vi "Lidar_Machine_etats.vi"() -> ()   [LabVIEW 2018]
uses:
  enum_etats_lidar.ctl
  <vilib>/Platform/TimedLoop/XDataNode/timing_clust.ctl
  <vilib>/Platform/TimedLoop/XDataNode/nitl_modes.ctl
  <vilib>/Platform/TimedLoop/XDataNode/wakeup.ctl
  enum_zone.ctl
  <vilib>/Platform/TimedLoop/XDataNode/XDataNode.xnode
  <vilib>/Platform/TimedLoop/XDataNode/XDNodeRunTimeDep.lvlib
panel:
  out "error boucle cadencé":errorcluster
  out "error boucle principale":errorcluster
  out "Espace libre":dbl[][](array[numeric])
  out "Zone 3":dbl[][](array[numeric])
  out "Zone 2":dbl[][](array[numeric])
  out "Timeout":bool=TRUE
  out "Selection de état":T1
  in  "stop boucle cadencé":bool
  out "Tableau lidar":dbl[][](array[numeric])=[[0.0, 1.0, 2.0, 3.0, 4.0, 5.0, 6.0, 7.0, 8.0, 9.0, 10.0, 11.0, 12.0, 13.0, 14.0, 15.0, 16.0, 17.0, 18.0, 19.0, 20.0, 21.0, 22.0, 23.0, 24.0, 25.0, 26.0, 27.0, 28.0, 29.0, 30.0, 31.0, 32.0, 33.0, 34.0, 35.0], [20.0, 15.0, 30.0, 31.0, 42.0, 50.0, 51.0, 60.0, 20.0, 15.0, 30.0, 31.0, 42.0, 50.0, 51.0, 60.0, 20.0, 15.0, 30.0, 31.0, 42.0, 50.0, 51.0, 60.0, 20.0, 15.0, 30.0, 31.0, 42.0, 50.0, 51.0, 60.0, 20.0, 15.0, 30.0, 31.0], [0.0, 0.0, 0.0, 0.0, 0.0, 0.0, 0.0, 0.0, 0.0, 0.0, 0.0, 0.0, 0.0, 0.0, 0.0, 0.0, 0.0, 0.0, 0.0, 0.0, 0.0, 0.0, 0.0, 0.0, 0.0, 0.0, 0.0, 0.0, 0.0, 0.0, 0.0, 0.0, 0.0, 0.0, 0.0, 0.0]]
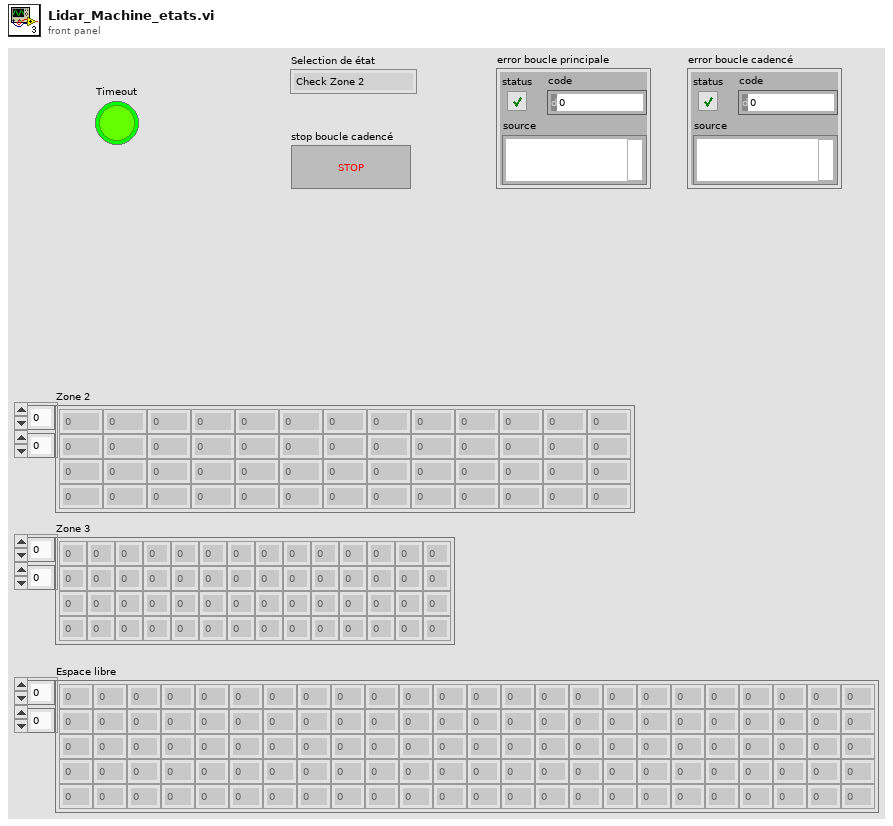
[diagram p1: front panel]
types:
  T1 = typedef "enum_etats_lidar.ctl" = enum16{"Check Zone 2", "Obstacle Zone 2", "Check Zone 3", "Obstacle Zone 3", "Avance", "Obstacle Timer", "Rescan 10s", "Check Zone 3 Bis", "Rotation new direction", "Rotation 180", "Timeout ?", "Arret complet", "Rotation new dir timer", "Rotation 180 timer"}
  T2 = typedef "enum_zone.ctl" = enum16{"Zone_2", "Zone_3", "Espace_libre", "Aucune"}
  T3 = typedef "XDNodeRunTimeDep.lvlib/timing_clust.ctl" = cluster{"Expected End [f-1]":u64, "Actual End [f-1]":u64, "Finished Late? [f-1]":bool, "Expected End [i-1]":u64, "Actual End [i-1]":u64, "Finished Late? [i-1]":bool, "Expected Start [i]":u64, "Actual Start [i]":u64, "Expected Start [f]":u64, "Actual Start [f]":u64, "Source Name":string, "Structure Name":string, "Period":i64, "Deadline":i64, "Offset":i64, "Start":i64, "Priority":i32, "Timeout":i32, "Mode":T4, "Wakeup Reason":T5, "Error":errorcluster, "Source Type":string, "Secondary Source Type":string, "Global End Time":u64, "Global Start Time":u64, "Frame Duration":u64, "Iteration Duration":u64, "Assigned CPU":i32, "I/O Scan Engine Mode":u32}
  T4 = typedef "XDNodeRunTimeDep.lvlib/nitl_modes.ctl" = enum32{"No Change", "Process missed periods, maintain original phase", "Discard missed periods, maintain original phase", "Process missed periods, ignore original phase", "Discard missed periods, ignore original phase"}
  T5 = typedef "XDNodeRunTimeDep.lvlib/wakeup.ctl" = enum32{"Normal", "Aborted", "Asynchronous wakeup", "Timing source error", "Timed loop error", "Timeout"}
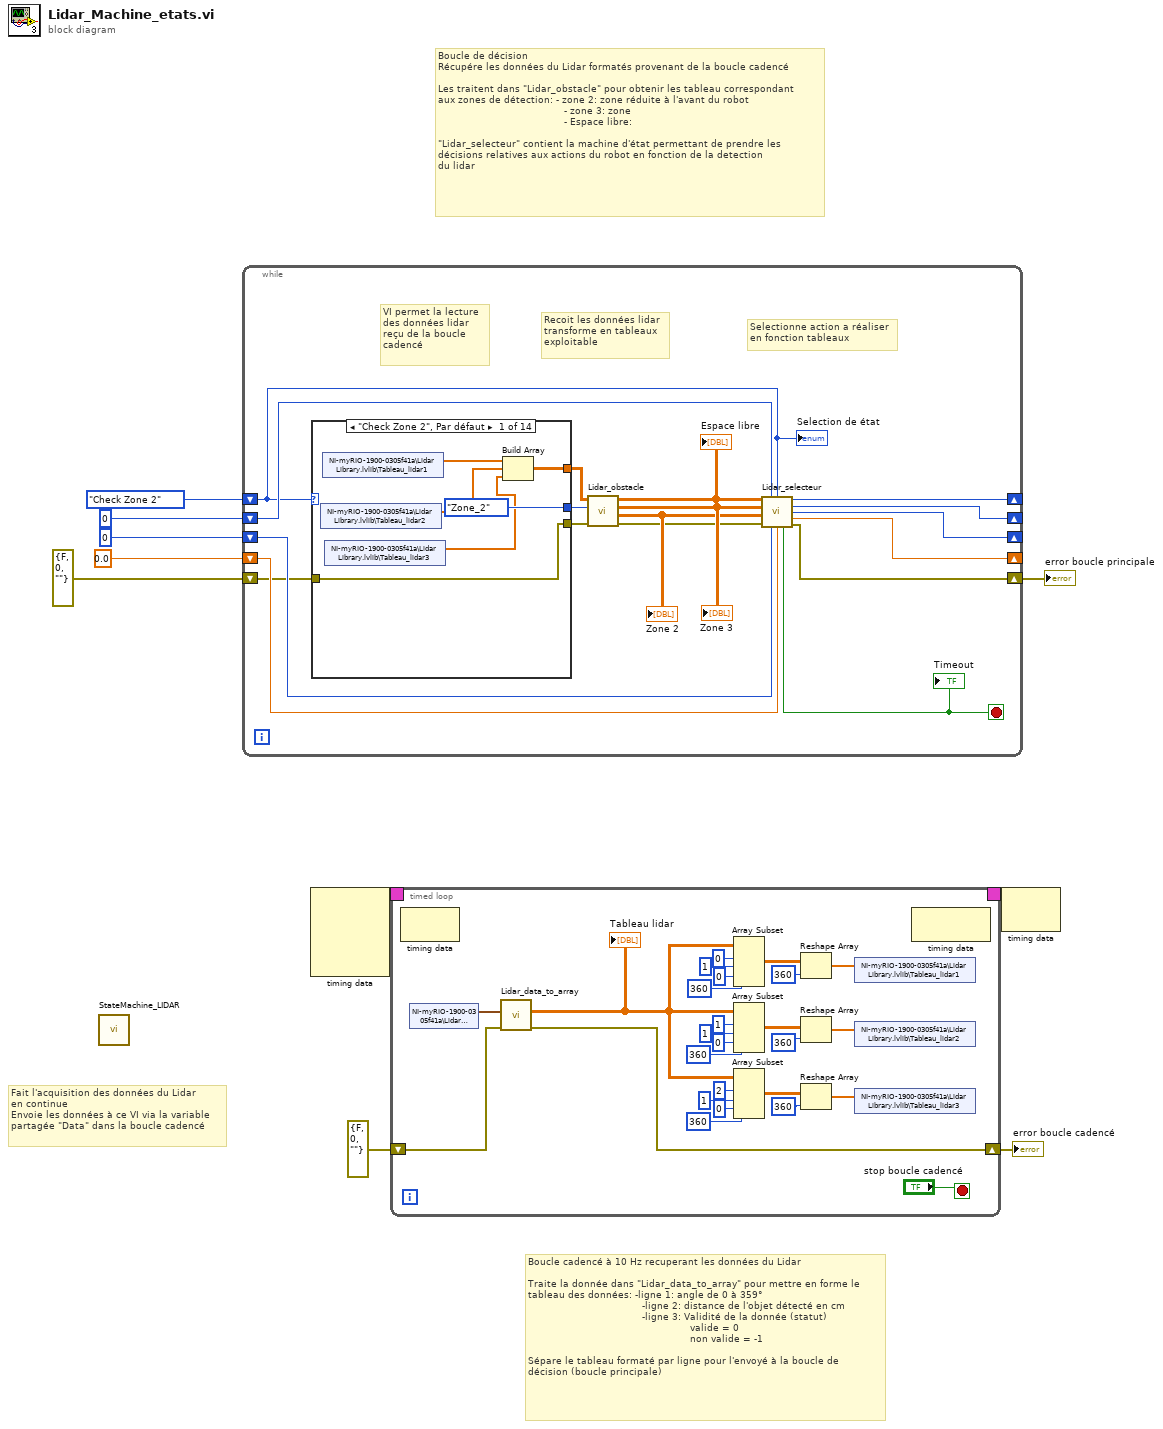
[diagram p0: block diagram]
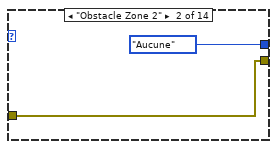
[diagram p2: hidden frame]
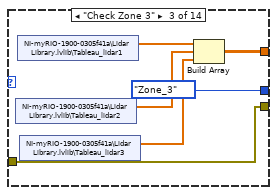
[diagram p3: hidden frame]
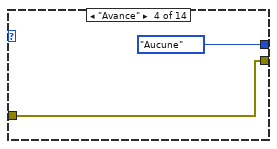
[diagram p4: hidden frame]
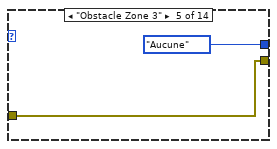
[diagram p5: hidden frame]
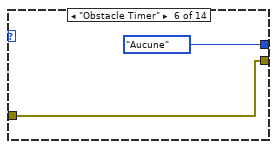
[diagram p6: hidden frame]
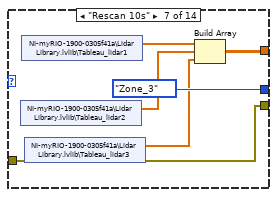
[diagram p7: hidden frame]
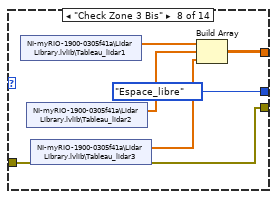
[diagram p8: hidden frame]
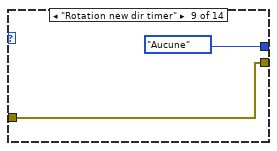
[diagram p9: hidden frame]
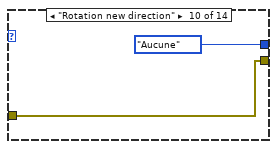
[diagram p10: hidden frame]
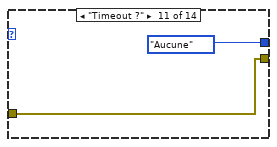
[diagram p11: hidden frame]
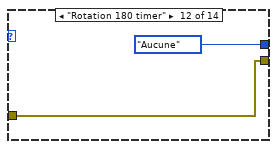
[diagram p12: hidden frame]
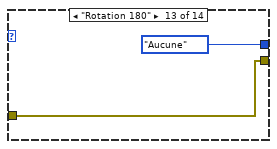
[diagram p13: hidden frame]
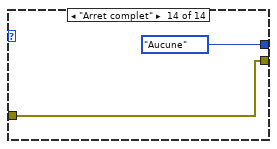
[diagram p14: hidden frame]
diagram:
  # "Boucle de décision\nRécupére les données du Lidar formatés provenant de la boucle cadencé\n\nLes traitent dans \"Lidar_obstacle\" pour obtenir les tableau correspondant \naux zones de détection: - zone 2: zone réduite à l'avant du robot\n                                          - zone 3: zone \n                                          - Espace libre: \n\n\"Lidar_selecteur\" contient la machine d'état permettant de prendre les\ndécisions relatives aux actions du robot en fonction de la detection\ndu lidar"
  # "Boucle cadencé à 10 Hz recuperant les données du Lidar\n\nTraite la donnée dans \"Lidar_data_to_array\" pour mettre en forme le\ntableau des données: -ligne 1: angle de 0 à 359°\n                                      -ligne 2: distance de l'objet détecté en cm\n                                      -ligne 3: Validité de la donnée (statut)\n                                                      valide = 0\n                                                      non valide = -1\n\nSépare le tableau formaté par ligne pour l'envoyé à la boucle de\ndécision (boucle principale)"
  # "Fait l'acquisition des données du Lidar\nen continue\nEnvoie les données à ce VI via la variable \npartagée \"Data\" dans la boucle cadencé"
  n1 = call "StateMachine_LIDAR.vi"() -> ()  [unwired: 12 in]
  n2 = while {
    shift-right: [w24] -> _
    shift-left: enum_etats_lidar."Check Zone 2" ("Selection de état") -> [w15]
    shift-right: [w22] -> _
    shift-left: u32 0 ("Timeout Count") -> [w23]
    shift-right: [w21] -> _
    shift-left: u32 0 ("Tick Count(mSec)") -> [w20]
    shift-right: [w18] -> _
    shift-left: 0.0 ("New Angle") -> [w19]
    shift-right: [w16] -> w2
    shift-left: errorcluster {"status"=FALSE, "code"=0, "source"=""} ("error out") -> [w13]
    stop <- w17 stop-if-true
    # "VI permet la lecture \ndes données lidar\nreçu de la boucle\ncadencé"
    # "Selectionne action a réaliser\nen fonction tableaux"
    # "Recoit les données lidar\ntransforme en tableaux \nexploitable"
    n3 = case shown="\"Check Zone 2\", Par défaut" w15 {
      tunnel: [enum_zone."Zone_2" ("Enum Zone") enum_zone."Aucune" ("Enum Zone") enum_zone."Zone_3" ("Enum Zone") enum_zone."Aucune" ("Enum Zone") enum_zone."Aucune" ("Enum Zone") enum_zone."Aucune" ("Enum Zone") enum_zone."Zone_3" ("Enum Zone") enum_zone."Espace_libre" ("Enum Zone") enum_zone."Aucune" ("Enum Zone") enum_zone."Aucune" ("Enum Zone") enum_zone."Aucune" ("Enum Zone") enum_zone."Aucune" ("Enum Zone") enum_zone."Aucune" ("Enum Zone") enum_zone."Aucune" ("Enum Zone")] -> w14
      tunnel: w13 -> [w33 w35 w41 w43 w45 w47 w53 w59 w61 w63 w65 w67 w69 w71]
      tunnel: [w33 w35 w41 w43 w45 w47 w53 w59 w61 w63 w65 w67 w69 w71] -> w12
      tunnel: [w29 _ w37 _ _ _ w52 w58 _ _ _ _ _ _] -> w11
      frame "Check Zone 2", Default {
        n4 = shared-variable "NI-myRIO-1900-0305f41a\\Lidar Library.lvlib\\Tableau_lidar2"() -> (w31:dbl[])  [unwired: 1 in, 1 out]
        n5 = shared-variable "NI-myRIO-1900-0305f41a\\Lidar Library.lvlib\\Tableau_lidar1"() -> (w32:dbl[])  [unwired: 1 in, 1 out]
        n6 = shared-variable "NI-myRIO-1900-0305f41a\\Lidar Library.lvlib\\Tableau_lidar3"() -> (w30:dbl[])  [unwired: 1 in, 1 out]
        n7 = Build Array(w32, w31, w30) -> (w29:dbl[][])
      }
      frame "Obstacle Zone 2" {
      }
      frame "Check Zone 3" {
        n8 = shared-variable "NI-myRIO-1900-0305f41a\\Lidar Library.lvlib\\Tableau_lidar2"() -> (w39:dbl[])  [unwired: 1 in, 1 out]
        n9 = shared-variable "NI-myRIO-1900-0305f41a\\Lidar Library.lvlib\\Tableau_lidar1"() -> (w40:dbl[])  [unwired: 1 in, 1 out]
        n10 = shared-variable "NI-myRIO-1900-0305f41a\\Lidar Library.lvlib\\Tableau_lidar3"() -> (w38:dbl[])  [unwired: 1 in, 1 out]
        n11 = Build Array(w40, w39, w38) -> (w37:dbl[][])
      }
      frame "Avance" {
      }
      frame "Obstacle Zone 3" {
      }
      frame "Obstacle Timer" {
      }
      frame "Rescan 10s" {
        n12 = shared-variable "NI-myRIO-1900-0305f41a\\Lidar Library.lvlib\\Tableau_lidar2"() -> (w50:dbl[])  [unwired: 1 in, 1 out]
        n13 = shared-variable "NI-myRIO-1900-0305f41a\\Lidar Library.lvlib\\Tableau_lidar1"() -> (w51:dbl[])  [unwired: 1 in, 1 out]
        n14 = shared-variable "NI-myRIO-1900-0305f41a\\Lidar Library.lvlib\\Tableau_lidar3"() -> (w49:dbl[])  [unwired: 1 in, 1 out]
        n15 = Build Array(w51, w50, w49) -> (w52:dbl[][])
      }
      frame "Check Zone 3 Bis" {
        n16 = shared-variable "NI-myRIO-1900-0305f41a\\Lidar Library.lvlib\\Tableau_lidar1"() -> (w57:dbl[])  [unwired: 1 in, 1 out]
        n17 = shared-variable "NI-myRIO-1900-0305f41a\\Lidar Library.lvlib\\Tableau_lidar2"() -> (w56:dbl[])  [unwired: 1 in, 1 out]
        n18 = shared-variable "NI-myRIO-1900-0305f41a\\Lidar Library.lvlib\\Tableau_lidar3"() -> (w55:dbl[])  [unwired: 1 in, 1 out]
        n19 = Build Array(w57, w56, w55) -> (w58:dbl[][])
      }
      frame "Rotation new dir timer" {
      }
      frame "Rotation new direction" {
      }
      frame "Timeout ?" {
      }
      frame "Rotation 180 timer" {
      }
      frame "Rotation 180" {
      }
      frame "Arret complet" {
      }
    }
    n20 = call "Lidar_obstacle.vi"("error in (no error)"=w12, "Enum Zone"=w14, "Tableau lidar"=w11) -> ("error out"=w25:errorcluster, "Zone 2"=w26:dbl[][], "Zone 3"=w27:dbl[][], "Espace libre"=w28:dbl[][])  [unwired: 5 in]
    "Zone 2" <- w26
    "Zone 3" <- w27
    "Espace libre" <- w28
    n21 = call "Lidar_selecteur.vi"("Espace dispo"=w28, "Timeout Count"=w23, "Enum état"=w15, "Zone 3"=w27, "Zone 2"=w26, "error in (no error)"=w25, "Tick Count(mSec)"=w20, "New Angle"=w19) -> ("Selection de état"=w24:T1, "Timeout Count"=w22:u32, "Tick Count(mSec)"=w21:u32, "New Angle"=w18:dbl, "Timeout"=w17:bool, "error out"=w16:errorcluster)  [unwired: 2 in]
    "Timeout" <- w17
    "Selection de état" <- w15
  }
  "error boucle principale" <- w2
  n22 = node-c288() -> (w5:T3)  [unwired: 4 in]
  n23 = timed-loop {
    timing: w5 -> [_]
    timing-out: [_] -> w4
    shift-right: [w73] -> w1
    shift-left: errorcluster {"status"=FALSE, "code"=0, "source"=""} ("error out") -> [w74]
    stop <- "stop boucle cadencé" stop-if-true
    n24 = node-c288() -> ()  [unwired: 1 in, 1 out]
    n25 = shared-variable "NI-myRIO-1900-0305f41a\\Lidar Library.lvlib\\Data"() -> (w97:cluster{"Angle":dbl, dbl}[])  [unwired: 1 in, 1 out]
    n26 = call "Lidar_data_to_array.vi"("error in"=w74, "Data"=w97) -> ("error out"=w73:errorcluster, "Tableau lidar formaté"=w96:dbl[][])  [unwired: 8 in]
    "Tableau lidar" <- w96
    n27 = Array Subset(array=w96, index (row)=0 ("index"), length (row)=1 ("length"), index (col)=0 ("index"), length (col)=360 ("length")) -> (w83:dbl[][])
    n28 = Array Subset(array=w96, index (row)=1 ("index"), length (row)=1 ("length"), index (col)=0 ("index"), length (col)=360 ("length")) -> (w78:dbl[][])
    n29 = Array Subset(array=w96, index (row)=2 ("index"), length (row)=1 ("length"), index (col)=0 ("index"), length (col)=360 ("length")) -> (w79:dbl[][])
    n30 = Reshape Array(w83, 360 ("dimension size")) -> (w77:dbl[])
    n31 = Reshape Array(w78, 360 ("dimension size")) -> (w76:dbl[])
    n32 = Reshape Array(w79, 360 ("dimension size")) -> (w75:dbl[])
    n33 = shared-variable "NI-myRIO-1900-0305f41a\\Lidar Library.lvlib\\Tableau_lidar1"(w77) -> ()  [unwired: 1 in, 1 out]
    n34 = shared-variable "NI-myRIO-1900-0305f41a\\Lidar Library.lvlib\\Tableau_lidar2"(w76) -> ()  [unwired: 1 in, 1 out]
    n35 = shared-variable "NI-myRIO-1900-0305f41a\\Lidar Library.lvlib\\Tableau_lidar3"(w75) -> ()  [unwired: 1 in, 1 out]
    n36 = node-c288() -> ()  [unwired: 1 in, 1 out]
  }
  "error boucle cadencé" <- w1
  n37 = node-c288(w4) -> ()  [unwired: 1 out]
